vi "Create Path (segments).vi"(5 "URI-Component.Path":refnum<class "URI-Component.Path.lvclass">, 8 "error in (no error)":errorcluster, 10 "base-path":string, 11 "Segments":string[](array[string])) -> (0 "error out":errorcluster, 2 "Path type":T1=enum."path-abempty", 3 "URI-Component.Path":refnum<class "URI-Component.Path.lvclass">)   [LabVIEW 2013, in "openURI.lvlib" / "URI-Component.Path.lvclass"]
uses:
  URI-Component.Path.lvclass
  path type -- enum.ctl
  URI-Component.Path.lvclass/URI-Component.Path.ctl
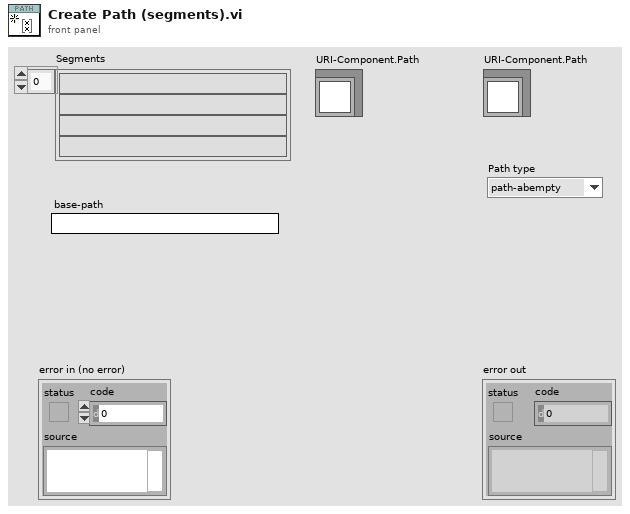
[diagram p1: front panel]
types:
  T1 = typedef "openURI.lvlib/URI-Component.Path.lvclass/path type -- enum.ctl" = enum16{"invalid", "path-abempty", "path-absolute", "path-noscheme", "path-rootless", "path-empty"}
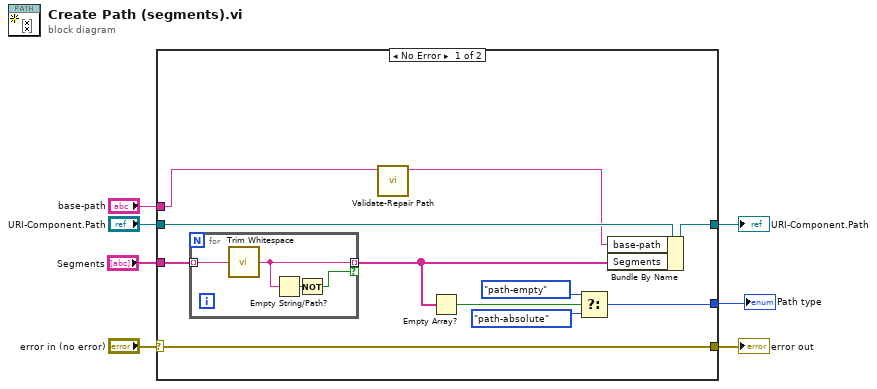
[diagram p0: block diagram]
diagram:
  n1 = case shown="No Error" "error in (no error)" {
    selector: "error in (no error)" -> [w18 w24]
    tunnel: [w18 w24] -> w6
    tunnel: [w16 w23] -> w4
    tunnel: "URI-Component.Path" -> [w17 w23]
    tunnel: "Segments" -> [w11 _]
    tunnel: [w12 _] -> w2
    tunnel: "base-path" -> [w9 _]
    frame No Error {
      n2 = for {
        tunnel: w11 -> [w22] mode=indexing
        tunnel: [w21] -> w10 mode=indexing if=w19
        n3 = call <vilib>:"Trim Whitespace.vi"("string"=w22) -> ("trimmed string"=w21:string)  [unwired: 1 in]
        n4 = Empty String/Path?(string/path=w21) -> (empty?=w20:bool)
        n5 = Not(x=w20) -> (.not. x?=w19:bool)
      }
      n6 = call "Validate-Repair Path.vi"("path in"=w9) -> ("path out"=w8:string)  [unwired: 7 in, 3 out]
      n7 = Empty Array?(array=w10) -> (empty?=w15:bool)
      n8 = Select(t=path_type_--_enum."path-empty" ("Path type"), s=w15, f=path_type_--_enum."path-absolute" ("Path type")) -> (s? t:f=w12:T1)
      n9 = Bundle By Name(cluster=w17, "base-path"=w8, "Segments"=w10) -> (w16:refnum<class "URI-Component.Path.lvclass">)
    }
    frame Error {
    }
  }
  "error out" <- w6
  "URI-Component.Path" <- w4
  "Path type" <- w2
